vi "lx.vi"() -> ()   [LabVIEW 2025]
uses:
  <vilib>/Instr/_visa.llb/VISA Configure Serial Port (Instr).vi
panel:
  out "read_buffer":string
  out "*(类型 *) &x":u32
  in  "baud rate":u16(ring) items=["9600"=9600, "115200"=65535]
  in  "exit":bool
  in  "serial_open":bool
  in  "serial":refnum<visa-resource-name> caption="VISA资源名称"
  out "serial_state":bool
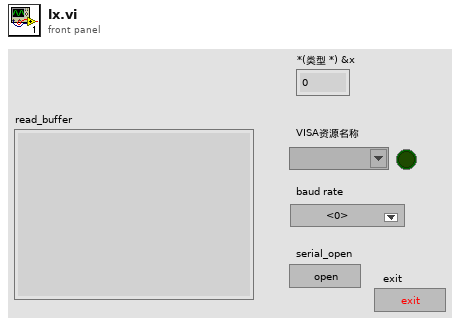
[diagram p1: front panel]
types:
  T1 = typedef "状态机.ctl" = enum16{"Init", "Wait", "send", "GetData", "deal", "Exit"}
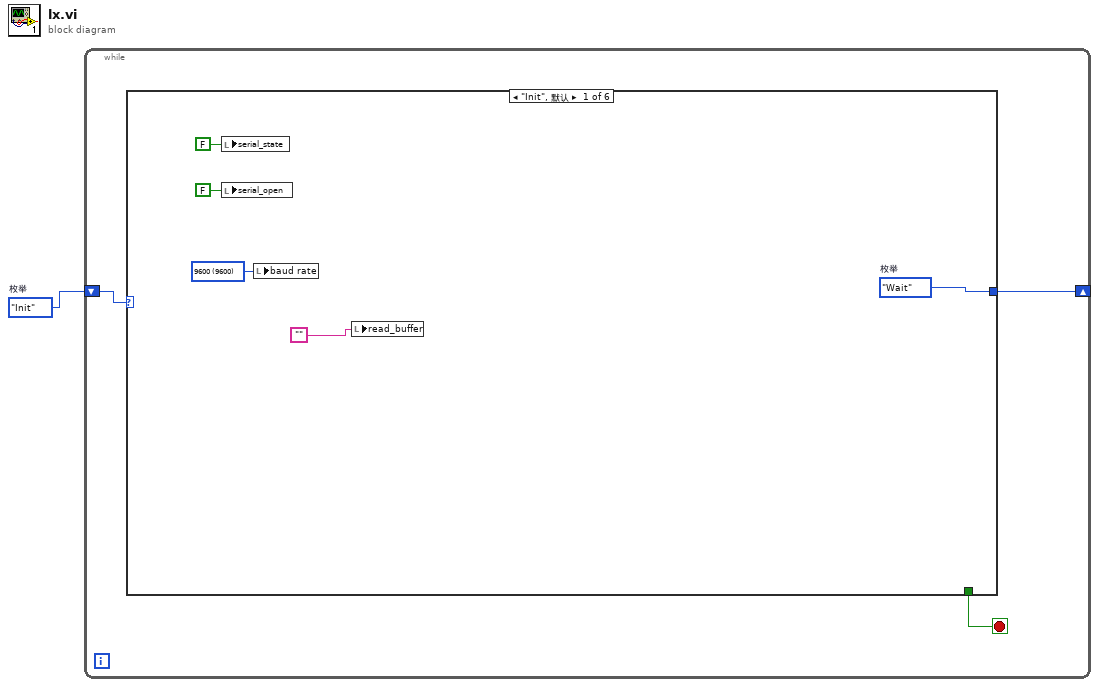
[diagram p0: block diagram]
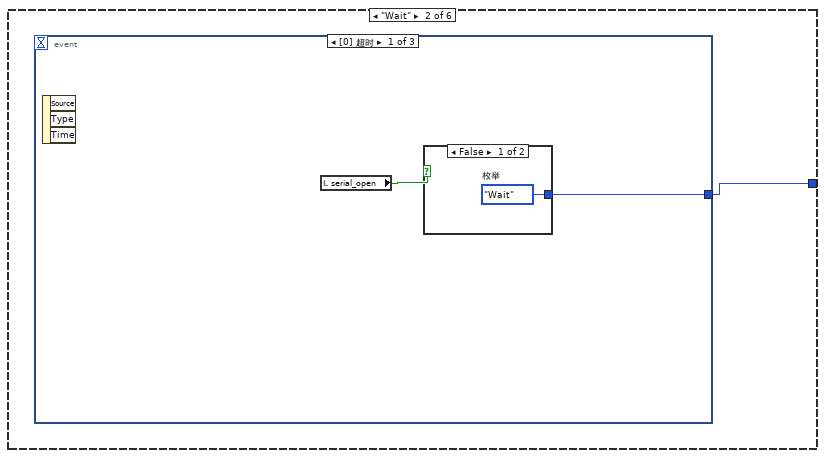
[diagram p2: hidden frame]
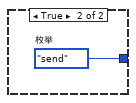
[diagram p3: hidden frame]
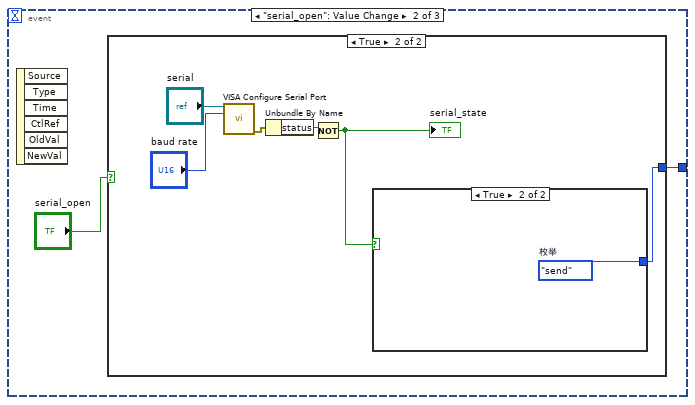
[diagram p4: hidden frame]
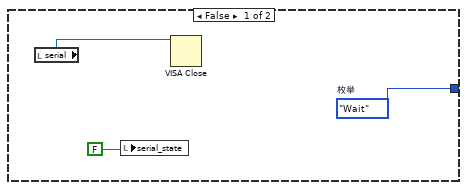
[diagram p5: hidden frame]
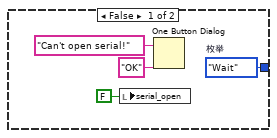
[diagram p6: hidden frame]
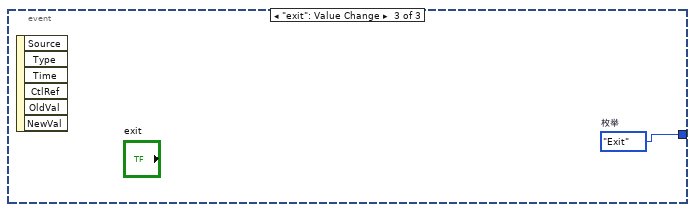
[diagram p7: hidden frame]
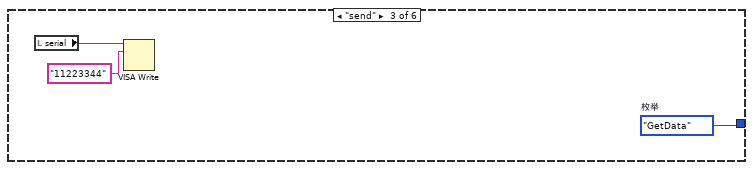
[diagram p8: hidden frame]
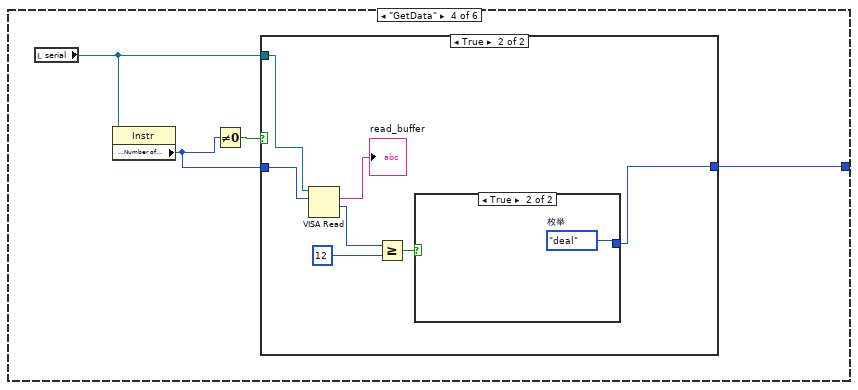
[diagram p9: hidden frame]
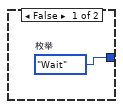
[diagram p10: hidden frame]
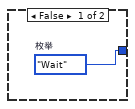
[diagram p11: hidden frame]
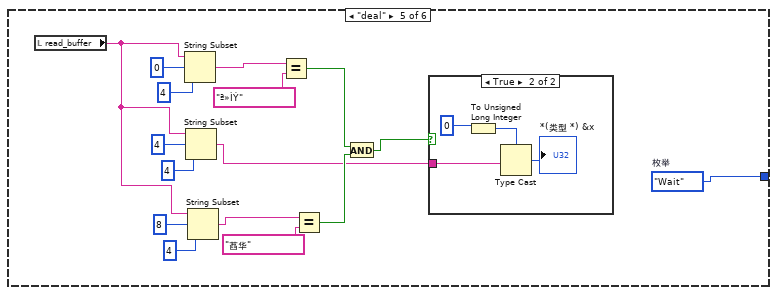
[diagram p12: hidden frame]
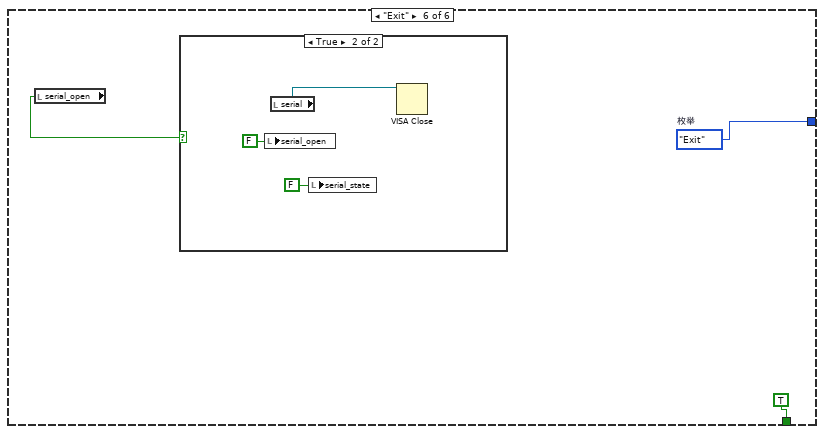
[diagram p14: hidden frame]
diagram:
  w1 = 状态机."Init"  # 枚举
  n1 = while {
    shift-right: [w3] -> _
    shift-left: w1 -> [w4]
    stop <- w2 stop-if-true
    n2 = case shown="\"Init\", 默认" w4 {
      tunnel: [w7 w10 w34 w35 w54 w71] -> w3
      tunnel: [_ _ _ _ _ TRUE ("exit")] -> w2
      frame "Init", Default {
        w5 = u16 9600 items=["9600"=9600, "115200"=65535] ("baud rate")
        w7 = 状态机."Wait"  # 枚举
        n3 = local write "serial_state"(FALSE ("布尔")) -> ()
        n4 = local write "serial_open"(FALSE ("serial_atate")) -> ()
        n5 = local write "baud rate"(w5) -> ()
        n6 = local write "read_buffer"("") -> ()
      }
      frame "Wait" {
        n7 = event shown="[0] 超时" {
          selector: _ -> [_ _ _]
          dyn-events: _ -> [_ _ _]
          timeout: _ -> [_ _ _]
          tunnel: [w11 w15 w31] -> w10
          event Timeout {
            n8 = event-data() -> ()  [unwired: 1 in, 3 out]
            n9 = local read "serial_open"() -> (w12:bool)
            n10 = case shown="False" w12 {
              tunnel: [w13 w14] -> w11
              frame False {
                w13 = 状态机."Wait"  # 枚举
              }
              frame True {
                w14 = 状态机."send"  # 枚举
              }
            }
          }
          event "serial_open": Value Change {
            n11 = event-data() -> ()  [unwired: 1 in, 6 out]
            n12 = case shown="True" "serial_open" {
              tunnel: [w17 w21] -> w15
              frame False {
                w17 = 状态机."Wait"  # 枚举
                n13 = local read "serial"() -> (w19:refnum<visa-resource-name>)
                n14 = local write "serial_state"(FALSE ("布尔")) -> ()
                n15 = VISA Close(VISA resource name=w19) -> ()  [unwired: 1 in, 1 out]
              }
              frame True {
                n16 = call-poly "VISA Configure Serial Port"("VISA resource name"="serial", "baud rate (9600)"="baud rate") -> ("error out"=w24:errorcluster)  [unwired: 12 in, 1 out]
                n17 = Unbundle By Name(w24) -> ("status"=w23:bool)
                n18 = Not(x=w23) -> (.not. x?=w22:bool)
                "serial_state" <- w22
                n19 = case shown="True" w22 {
                  tunnel: [w26 w30] -> w21
                  frame False {
                    w26 = 状态机."Wait"  # 枚举
                    n20 = local write "serial_open"(FALSE ("serial_atate")) -> ()
                    n21 = One Button Dialog(message="Can't open serial!" ("消息"), button name ("OK")="OK" ("按钮名称（“确定”）")) -> ()  [unwired: 1 out]
                  }
                  frame True {
                    w30 = 状态机."send"  # 枚举
                  }
                }
              }
            }
          }
          event "exit": Value Change {
            w31 = 状态机."Exit"  # 枚举
            n22 = event-data() -> ()  [unwired: 1 in, 6 out]
          }
        }
      }
      frame "send" {
        w34 = 状态机."GetData"  # 枚举
        n23 = local read "serial"() -> (w33:refnum<visa-resource-name>)
        n24 = VISA Write(VISA resource name=w33, write buffer="11223344" ("写入缓冲区")) -> ()  [unwired: 1 in, 3 out]
      }
      frame "GetData" {
        n25 = local read "serial"() -> (w38:refnum<visa-resource-name>)
        n26 = property class="Instr"(reference=w38) -> ("Serial Settings:Number of Bytes at Serial Port"=w36:u32)  [unwired: 1 in, 2 out]
        n27 = Not Equal To 0?(x=w36) -> (x != 0?=w37:bool)
        n28 = case shown="True" w37 {
          tunnel: w38 -> [_ w46]
          tunnel: w36 -> [_ w45]
          tunnel: [w39 w41] -> w35
          frame False {
            w39 = 状态机."Wait"  # 枚举
          }
          frame True {
            n29 = VISA Read(VISA resource name=w46, byte count=w45) -> (read buffer=→"read_buffer":string, return count=w44:u32)  [unwired: 1 in, 2 out]
            n30 = Greater Or Equal?(x=w44, y=u32 12) -> (x >= y?=w42:bool)
            n31 = case shown="True" w42 {
              tunnel: [w47 w48] -> w41
              frame False {
                w47 = 状态机."Wait"  # 枚举
              }
              frame True {
                w48 = 状态机."deal"  # 枚举
              }
            }
          }
        }
      }
      frame "deal" {
        w54 = 状态机."Wait"  # 枚举
        n32 = local read "read_buffer"() -> (w49:string)
        n33 = String Subset(string=w49, offset (0)=0 ("偏移量(0)"), length (rest)=4 ("长度（剩余）")) -> (substring=w58:string)
        n34 = String Subset(string=w49, offset (0)=4 ("偏移量(0)"), length (rest)=4 ("长度（剩余）")) -> (substring=w50:string)
        n35 = String Subset(string=w49, offset (0)=8 ("偏移量(0)"), length (rest)=4 ("长度（剩余）")) -> (substring=w55:string)
        n36 = Equal?(x=w58, y="ª»ÌÝ") -> (x = y?=w53:bool)
        n37 = Equal?(x=w55, y="萏华") -> (x = y?=w52:bool)
        n38 = And(x=w53, y=w52) -> (x .and. y?=w51:bool)
        n39 = case shown="True" w51 {
          tunnel: w50 -> [_ w68]
          frame False {
          }
          frame True {
            n40 = To Unsigned Long Integer(number=0) -> (unsigned 32bit integer=w65:u32)
            n41 = Type Cast(type=w65, x=w68) -> (*(type *) &x=→"*(类型 *) &x":u32)
          }
        }
      }
      frame "Exit" {
        w71 = 状态机."Exit"  # 枚举
        n42 = local read "serial_open"() -> (w69:bool)
        n43 = case shown="True" w69 {
          frame False {
          }
          frame True {
            n44 = local write "serial_open"(FALSE ("serial_state")) -> ()
            n45 = local read "serial"() -> (w73:refnum<visa-resource-name>)
            n46 = local write "serial_state"(FALSE ("serial_state")) -> ()
            n47 = VISA Close(VISA resource name=w73) -> ()  [unwired: 1 in, 1 out]
          }
        }
      }
    }
  }
